vi "NIDAQmx Logic.vi"(8 "error in (no error)":errorcluster, 9 "channel":string, 10 "Session Factory in":refnum<class "Session Factory.lvclass">, 11 "Measurement Configuration":T2) -> (0 "error out":errorcluster, 3 "Measurement Results":T1)   [LabVIEW 2021, in "NIDAQmxMeasurement.lvlib"]
doc: "This example demonstrates how to measure a finite single frequency sample. It uses implicit timing, \nwhich means that a sample is acquired for every period of your input signal. The Set Channel Property \n(CI Frequency Input Terminal and CI Frequency Measurement) helps specify the input terminal of \nthe signal to measure and the duration for measuring the signal frequency.\n\nFor more information, see the DAQmx \nexample: <examples>\\DAQmx\\Counter Input\\Counter - Read Pulse Width and Frequency (Finite).vi"
uses:
  NIDAQmxMeasurement.lvlib
  Measurement Configuration.ctl
  Measurement Results.ctl
  <vilib>/Plug-In SDKs/Sessions/niDAQmx/Session Factory/Session Factory.lvclass
  <vilib>/Plug-In SDKs/Sessions/niDAQmx/Session Factory/Client Wrapper Functions/niDAQmx Get Task Property (Name).vi
  <vilib>/Plug-In SDKs/Sessions/niDAQmx/Session Factory/Client Wrapper Functions/niDAQmx Create Virtual Channel (CI Frequency).vi
  <vilib>/Plug-In SDKs/Sessions/niDAQmx/Session Factory/Client Wrapper Functions/niDAQmx Set Channel Property (CI Frequency Input Terminal).vi
  <vilib>/Plug-In SDKs/Sessions/niDAQmx/Session Factory/Client Wrapper Functions/niDAQmx Set Channel Property (CI Frequency Measurement Time).vi
  <vilib>/Plug-In SDKs/Sessions/niDAQmx/Session Factory/Client Wrapper Functions/niDAQmx Timing (Implicit).vi
  <vilib>/Plug-In SDKs/Sessions/niDAQmx/Session Factory/Client Wrapper Functions/niDAQmx Get Channel Property (CI Frequency Measurement Time).vi
  <vilib>/Plug-In SDKs/Sessions/niDAQmx/Session Factory/Client Wrapper Functions/niDAQmx Read (Counter DBL 1Chan 1Samp).vi
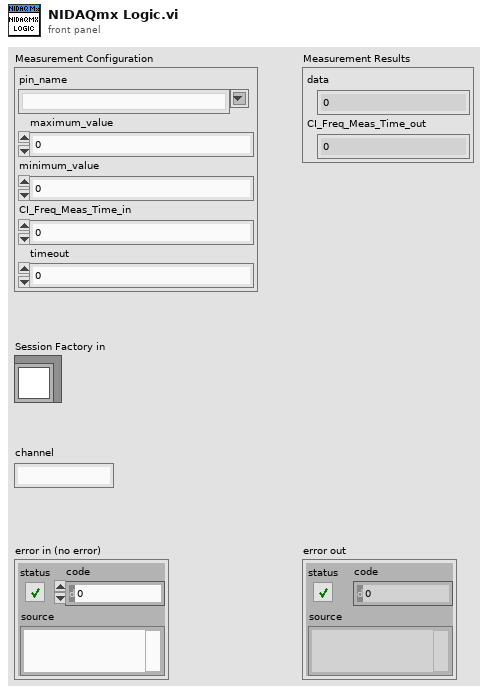
[diagram p1: front panel]
types:
  T1 = typedef "NIDAQmxMeasurement.lvlib/Measurement Results.ctl" = cluster{"data":dbl, "CI_Freq_Meas_Time_out":dbl}
  T2 = typedef "NIDAQmxMeasurement.lvlib/Measurement Configuration.ctl" = cluster{"pin_name":string, "maximum_value":dbl, "minimum_value":dbl, "CI_Freq_Meas_Time_in":dbl, "timeout":dbl}
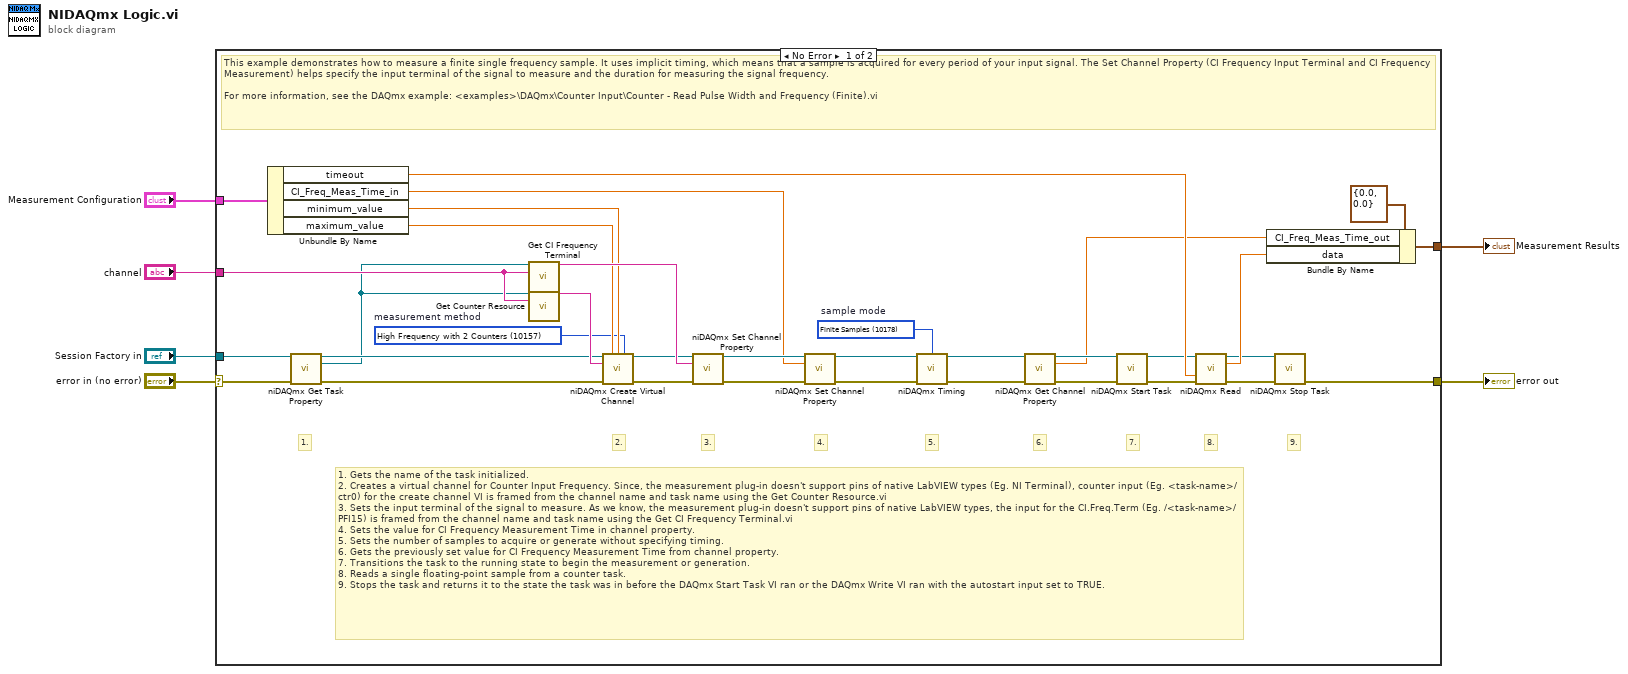
[diagram p0: block diagram]
diagram:
  n1 = case shown="No Error" "error in (no error)" {
    selector: "error in (no error)" -> [w19 w41]
    tunnel: "Measurement Configuration" -> [w40 _]
    tunnel: [w39 _] -> w5
    tunnel: [w13 w41] -> w4
    tunnel: "Session Factory in" -> [w16 _]
    tunnel: "channel" -> [w20 _]
    frame No Error {
      w7 = 10157 items=["Low Frequency with 1 Counter"=10105, "High Frequency with 2 Counters"=10157, "Large Range with 2 Counters"=10205, "Dynamic Averaging"=16065]  # measurement method
      w32 = 10178 items=["Finite Samples"=10178, "Continuous Samples"=10123, "Hardware Timed Single Point"=12522]  # sample mode
      # "9."
      # "1. Gets the name of the task initialized.\n2. Creates a virtual channel for Counter Input Frequency. Since, the measurement plug-in doesn't support pins of native LabVIEW types (Eg. NI Terminal), counter input (Eg. <task-name>/ctr0) for the create channel VI is framed from the channel name and task name using the Get Counter Resource.vi\n3. Sets the input terminal of the signal to measure. As we know, the measurement plug-in doesn't support pins of native LabVIEW types, the input for the CI.Freq.Term (Eg. /<task-name>/PFI15) is framed from the channel name and task name using the Get CI Frequency Terminal.vi\n4. Sets the value for CI Frequency Measurement Time in channel property. \n5. Sets the number of samples to acquire or generate without specifying timing.\n6. Gets the previously set value for CI Frequency Measurement Time from channel property. \n7. Transitions the task to the running state to begin the measurement or generation.\n8. Reads a single floating-point sample from a counter task. \n9. Stops the task and returns it to the state the task was in before the DAQmx Start Task VI ran or the DAQmx Write VI ran with the autostart input set to TRUE."
      # "8."
      # "7."
      # "6."
      # "5."
      # "4."
      # "3."
      # "2."
      # "1."
      # "This example demonstrates how to measure a finite single frequency sample. It uses implicit timing, which means that a sample is acquired for every period of your input signal. The Set Channel Property (CI Frequency Input Terminal and CI Frequency Measurement) helps specify the input terminal of the signal to measure and the duration for measuring the signal frequency.\n\nFor more information, see the DAQmx example: <examples>\\DAQmx\\Counter Input\\Counter - Read Pulse Width and Frequency (Finite).vi"
      n2 = Unbundle By Name(w40) -> ("timeout"=w36:dbl, "CI_Freq_Meas_Time_in"=w21:dbl, "minimum_value"=w33:dbl, "maximum_value"=w14:dbl)
      n3 = call-poly <vilib>:"niDAQmx Get Task Property.vi"("task in"=w16, "error in"=w19) -> ("task out"=w17:refnum<class "Session Factory.lvclass">, "Name"=w15:refnum<k21>, "error out"=w18:errorcluster)  [unwired: 11 in]
      n4 = call "Get CI Frequency Terminal.vi"("Task Name"=w15, "channel"=w20) -> ("CI.Freq.Term"=w35:tag)  [unwired: 13 in]
      n5 = call "Get Counter Resource.vi"("Task Name"=w15, "channel"=w20) -> ("counter"=w34:tag)  [unwired: 13 in]
      n6 = call-poly <vilib>:"niDAQmx Create Virtual Channel.vi"("task in"=w17, "maximum value"=w14, "minimum value"=w33, "measurement method"=w7, "counter"=w34, "error in"=w18) -> ("task out"=w27:refnum<class "Session Factory.lvclass">, "error out"=w26:errorcluster)  [unwired: 8 in]
      n7 = call-poly <vilib>:"niDAQmx Set Channel Property.vi"("task in"=w27, "CI.Freq.Term"=w35, "error in"=w26) -> ("task out"=w23:refnum<class "Session Factory.lvclass">, "error out"=w25:errorcluster)  [unwired: 11 in]
      n8 = call-poly <vilib>:"niDAQmx Set Channel Property.vi"("task in"=w23, "CI.Freq.MeasTime"=w21, "error in"=w25) -> ("task out"=w22:refnum<class "Session Factory.lvclass">, "error out"=w24:errorcluster)  [unwired: 11 in]
      n9 = call-poly <vilib>:"niDAQmx Timing.vi"("task/channels in"=w22, "samples per channel"=w32, "error in"=w24) -> ("task out"=w10:refnum<class "Session Factory.lvclass">, "error out"=w12:errorcluster)  [unwired: 11 in]
      n10 = call-poly <vilib>:"niDAQmx Get Channel Property.vi"("task in"=w10, "error in"=w12) -> ("task out"=w9:refnum<class "Session Factory.lvclass">, "CI.Freq.MeasTime"=w8:dbl, "error out"=w11:errorcluster)  [unwired: 11 in]
      n11 = call <vilib>:"niDAQmx Start Task.vi"("task/channels in"=w9, "error in"=w11) -> ("task out"=w30:refnum<class "Session Factory.lvclass">, "error out"=w28:errorcluster)  [unwired: 12 in]
      n12 = call-poly <vilib>:"niDAQmx Read.vi"("task in"=w30, "timeout"=w36, "error in"=w28) -> ("task out"=w31:refnum<class "Session Factory.lvclass">, "data"=w38:dbl, "error out"=w29:errorcluster)  [unwired: 10 in]
      n13 = Bundle By Name(cluster=T1 {"data"=0.0, "CI_Freq_Meas_Time_out"=0.0} ("Measurement Results"), "CI_Freq_Meas_Time_out"=w8, "data"=w38) -> (w39:T1)
      n14 = call <vilib>:"niDAQmx Stop Task.vi"("task/channels in"=w31, "error in"=w29) -> ("error out"=w13:errorcluster)  [unwired: 12 in, 1 out]
    }
    frame Error {
    }
  }
  "Measurement Results" <- w5
  "error out" <- w4
